vi "wiringPiSPIxDataRW.vi"(8 "error in (no error)":errorcluster, 9 "len":i32, 10 "data in":u8[](array[numeric]), 11 "SPI Device":T1) -> (0 "error out":errorcluster, 1 "return":i32, 2 "data out":u8[](array[numeric]), 3 "SPI Device out":T1)   [LabVIEW 2025, in "wiringPi.lvlib"]
doc: "<b>_______________________________________________________________</b>\n** Author: Juan José Villacorta\n** LabVIEW wrapper for C library <b> wiringPi </b>,\n** https://github.com/WiringPi/WiringPi\n<b>_______________________________________________________________</b>\n\n/*\n * wiringPiSPIDataRW:\n * Write and Read a block of data over the SPI bus.\n * Note the data ia being read into the transmit buffer, so will\n * overwrite it!\n * This is also a full-duplex operation.\n *********************************************************************************\n */"
uses:
  wiringPi.lvlib
  Type Defs/SPI Device.ctl
  Type Defs/SPI Dev.ctl
  Type Defs/SPI Channel.ctl
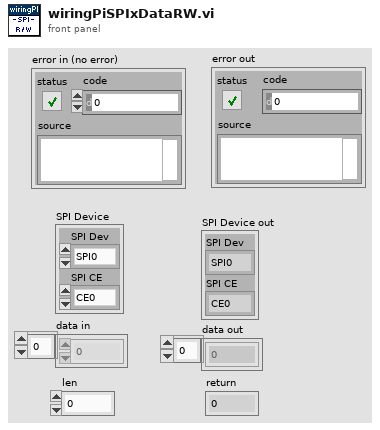
[diagram p1: front panel]
types:
  T1 = typedef "wiringPi.lvlib/SPI Device.ctl" = cluster{"SPI Dev":T2, "SPI CE":T3}
  T2 = typedef "wiringPi.lvlib/SPI Dev.ctl" = enum32{"SPI0", "SPI1"}
  T3 = typedef "wiringPi.lvlib/SPI Channel.ctl" = enum32{"CE0", "CE1", "CE2"}
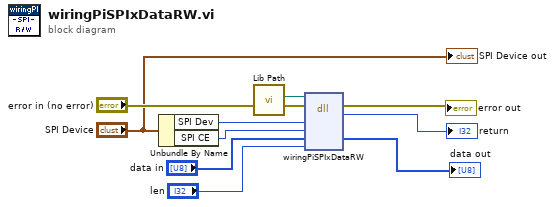
[diagram p0: block diagram]
diagram:
  n1 = Unbundle By Name("SPI Device") -> ("SPI Dev"=w8:T2, "SPI CE"=w7:T3)
  n2 = call "Lib Path.vi"() -> ("path out"=w2:path)  [unwired: 11 in]
  n3 = dll-call lib="libLVwiringPI.so" fn="wiringPiSPIxDataRW"(path in=w2, error in="error in (no error)", "number"=w8, "channel"=w7, "data"="data in", "len"="len") -> (error out=→"error out":errorcluster, "return type"=→"return":i32, "data"=→"data out":u8[])  [unwired: 4 in, 1 out]
  "SPI Device out" <- "SPI Device"
